vi "draw.vi"(0 "reference":refnum<class "NoteNode.lvclass">, 1 "graphics":refnum<class "Graphics.lvclass">, 5 "error in (no error)":errorcluster) -> (14 "reference out":refnum<class "NoteNode.lvclass">, 19 "error out":errorcluster)   [LabVIEW 2020, in "NoteNode.lvclass"]
doc: "public void draw(Graphics2D g2)"
uses:
  <resource>/Framework/Providers/Open_GDS/UML/NoteNode_class/NoteNode.lvclass
  C:/Program Files (x86)/National Instruments/LabVIEW 2020/resource/Framework/Providers/Open_GDS/UML/RectangularNode_class/RectangularNode.lvclass
  <resource>/Framework/Providers/Open_GDS/UML/Graphics_class/Graphics.lvclass
  <resource>/Framework/Providers/Open_GDS/UML/MultiLineString_class/MultiLineString.lvclass
  <resource>/Framework/Providers/Open_GDS/UML/RectangularNode_class/RectangularNode.lvclass
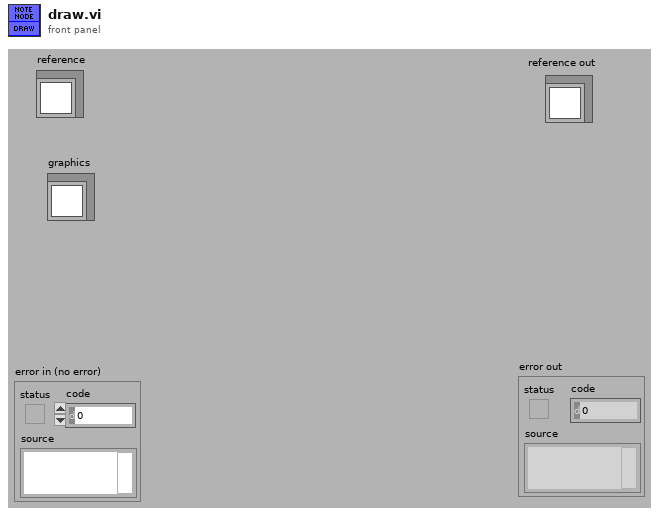
[diagram p1: front panel]
types:
  T1 = typedef "NoteNode.lvclass/ObjectAttributes.ctl" = cluster{"DEFAULT_WIDTH":i32, "DEFAULT_HEIGHT":i32, "DEFAULT_COLOR":u32, "FOLD_X":i32, "FOLD_Y":i32, "color":u32, "text":refnum<class "MultiLineString.lvclass">, "pointNodes":refnum<class "AbstractNode.lvclass">[]}
  T2 = typedef "RectangularNode.lvclass/ObjectAttributes.ctl" = cluster{"bounds":T3}
  T3 = typedef "Rectangle Rectangle2D.ctl" = cluster{"x":dbl, "y":dbl, "width":dbl, "height":dbl}
  T4 = typedef "Point Point2D.ctl" = cluster{"x":dbl, "y":dbl}
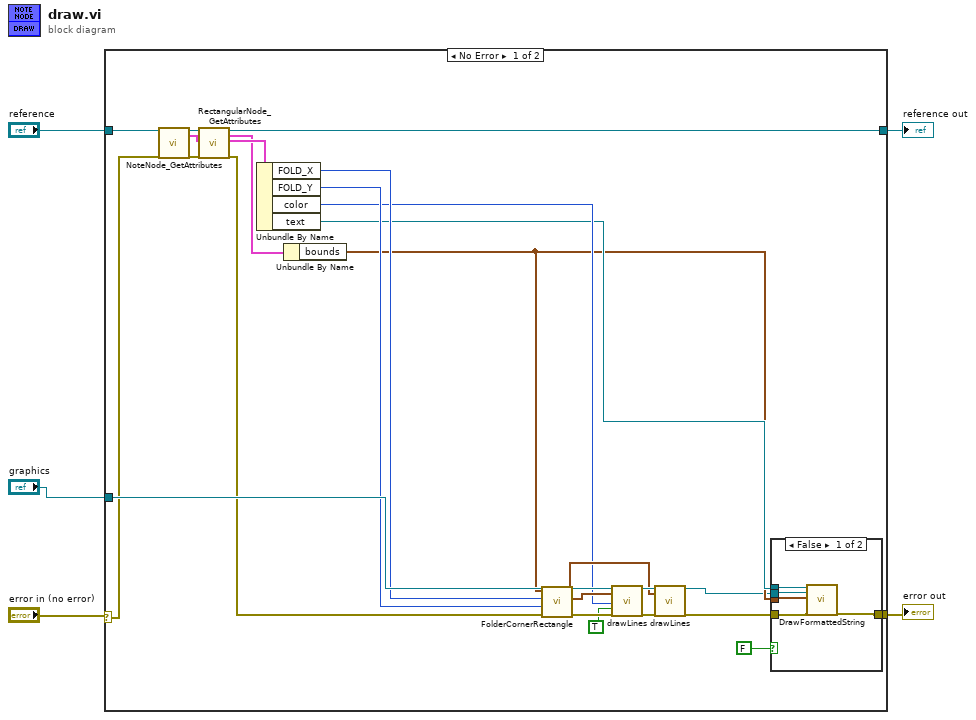
[diagram p0: block diagram]
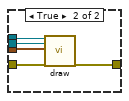
[diagram p2: hidden frame]
diagram:
  n1 = case shown="No Error" "error in (no error)" {
    selector: "error in (no error)" -> [w15 w40]
    tunnel: "reference" -> [w29 w41]
    tunnel: [w28 w40] -> w4
    tunnel: [w7 w41] -> w3
    tunnel: "graphics" -> [w27 _]
    frame No Error {
      n2 = call <resource>:"NoteNode_GetAttributes.vi"("reference in"=w29, "error in (no error)"=w15) -> ("reference out"=w10:refnum<class "NoteNode.lvclass">, "Data"=w11:T1, "error out"=w9:errorcluster)  [unwired: 1 in, 14 out]
      n3 = call <resource>:"RectangularNode_GetAttributes.vi"("reference in"=w10, "error in (no error)"=w9) -> ("reference out"=w7:refnum<class "NoteNode.lvclass">, "Data"=w6:T2, "error out"=w8:errorcluster)  [unwired: 14 in, 1 out]
      n4 = Unbundle By Name(w11) -> ("FOLD_X"=w26:i32, "FOLD_Y"=w25:i32, "color"=w20:u32, "text"=w19:refnum<class "MultiLineString.lvclass">)
      n5 = Unbundle By Name(w6) -> ("bounds"=w14:T3)
      n6 = call <resource>:"FolderCornerRectangle.vi"("error out 2"=w8, "FOLD_Y"=w25, "FOLD_X"=w26, "bounds"=w14) -> ("error out"=w17:errorcluster, "Array 2"=w24:T4[], "Array"=w21:T4[])  [unwired: 5 out]
      n7 = call <resource>:"drawLines.vi"("reference"=w27, "points"=w24, "color(if not used=default color)"=w20, "fill?(F)"=TRUE, "error in (no error)"=w17) -> ("reference out"=w23:refnum<class "Graphics.lvclass">, "error out"=w22:errorcluster)  [unwired: 2 in, 11 out]
      n8 = call <resource>:"drawLines.vi"("reference"=w23, "points"=w21, "error in (no error)"=w22) -> ("reference out"=w13:refnum<class "Graphics.lvclass">, "error out"=w18:errorcluster)  [unwired: 4 in, 11 out]
      n9 = case shown="False" FALSE {
        tunnel: [w32 w39] -> w28
        tunnel: w19 -> [w34 w38]
        tunnel: w18 -> [w33 w37]
        tunnel: w14 -> [w30 w36]
        tunnel: w13 -> [w31 w35]
        frame False {
          n10 = call-dynamic "DrawFormattedString.vi"("reference"=w34, "graphics"=w31, "bounds"=w30, "error in (no error)"=w33) -> ("error out"=w32:errorcluster)  [unwired: 14 in, 1 out]
        }
        frame True {
          n11 = call-dynamic "draw.vi"("reference"=w38, "graphics"=w35, "bounds"=w36, "error in (no error)"=w37) -> ("error out"=w39:errorcluster)  [unwired: 14 in, 1 out]
        }
      }
    }
    frame Error {
    }
  }
  "reference out" <- w3
  "error out" <- w4
